vi "RDV-handle-Impedance.vi"(5 "Use ignore list (false)":bool, 8 "error in (no error)":errorcluster, 11 "RDV-Reflection_Data_viewer in":refnum<class "RDV-Reflection_Data_viewer.lvclass">) -> (0 "error out":errorcluster, 3 "RDV-Reflection_Data_viewer out":refnum<class "RDV-Reflection_Data_viewer.lvclass">)   [LabVIEW 2020, in "RDV-Reflection_Data_viewer.lvclass"]
doc: "Computes the impedance of all data in the viewer's map with RDC-Lin-Calc_Impedance2 and adds the results to the map."
uses:
  RDV-Reflection_Data_viewer.lvclass
  Computation/RDC-Reflection_Data_Computation.lvlib
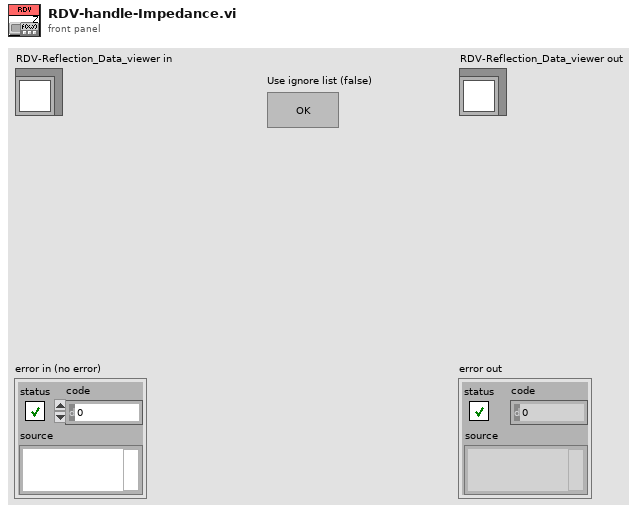
[diagram p1: front panel]
types:
  T1 = typedef "RFH-Reflection_File_Handler.lvlib/RFH-common_data_format.ctl" = cluster{"Frequency":dbl[], "Reflection'":dbl[], "Reflection''":dbl[], "Permativity'":dbl[], "Permativity''":dbl[], "Conductivity":dbl[], "Loss Tangent":dbl[], "Resistance":dbl[], "Reactance":dbl[]}
  T2 = typedef "RDV-Reflection_Data_viewer.lvclass/RDV-DATA_MAP_CLUST.ctl" = cluster{"filename w/ ext":string, "Common Format":T1}
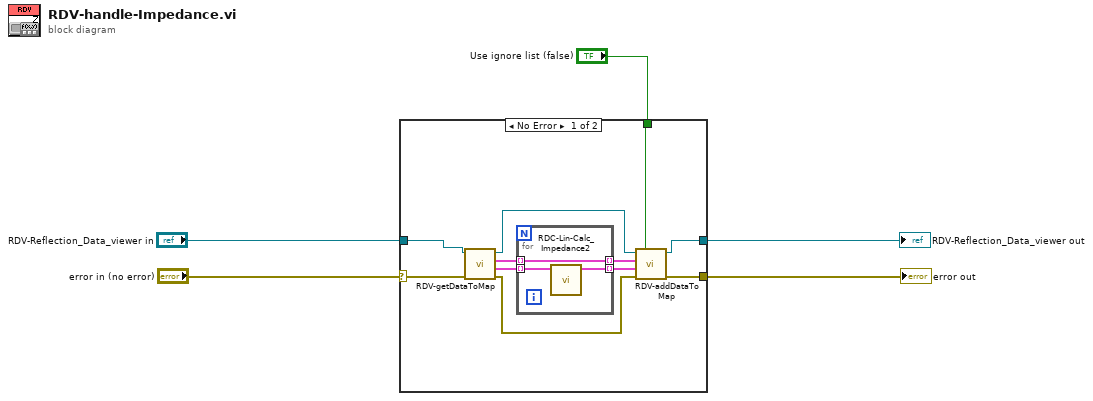
[diagram p0: block diagram]
diagram:
  n1 = case shown="No Error" "error in (no error)" {
    selector: "error in (no error)" -> [w6 w21]
    tunnel: [w7 w21] -> w4
    tunnel: [w8 w20] -> w2
    tunnel: "RDV-Reflection_Data_viewer in" -> [w9 w20]
    tunnel: "Use ignore list (false)" -> [w10 _]
    frame No Error {
      n2 = call "RDV-getDataToMap.vi"("error in (no error)"=w6, "RDV-Reflection_Data_viewer in"=w9) -> ("error out"=w14:errorcluster, "data"=w15:T1[], "all data"=w16:cluster{"key":string, "data":T2}[], "RDV-Reflection_Data_viewer out"=w13:refnum<class "RDV-Reflection_Data_viewer.lvclass">)  [unwired: 6 in]
      n3 = for {
        tunnel: w16 -> [w17] mode=indexing
        tunnel: w15 -> [w19] mode=indexing
        tunnel: [w18] -> w11 mode=indexing
        tunnel: [w17] -> w12 mode=indexing
        n4 = call "RDC-Lin-Calc_Impedance2.vi"("input cluster"=w19) -> ("Output cluster"=w18:T1)  [unwired: 9 in, 1 out]
      }
      n5 = call "RDV-addDataToMap.vi"("Use ignore list (false)"=w10, "error in (no error)"=w14, "data"=w11, "all data"=w12, "RDV-Reflection_Data_viewer in"=w13) -> ("error out"=w7:errorcluster, "RDV-Reflection_Data_viewer out"=w8:refnum<class "RDV-Reflection_Data_viewer.lvclass">)  [unwired: 5 in]
    }
    frame Error {
    }
  }
  "error out" <- w4
  "RDV-Reflection_Data_viewer out" <- w2
